vi "Configure Session.vi"(8 "error in":errorcluster, 11 "Plugin in":refnum<class "Nominal-TDMS-Upload.lvclass">) -> (0 "error out":errorcluster, 3 "Plugin out":refnum<class "Nominal-TDMS-Upload.lvclass">)   [LabVIEW 2026, in "Nominal-TDMS-Upload.lvlib" / "Nominal-TDMS-Upload.lvclass"]
uses:
  Nominal-TDMS-Upload.lvclass
  C:/Program Files/National Instruments/LabVIEW 2026/vi.lib/FlexLogger/SDK/PluginSDK.lvlibp/PEFClasses/SDK/Plugin/Plugin.lvclass
  stream reference data.ctl
  <vilib>/Nominal/Nominal IO Client/lv_src/Nominal Client/Nominal Client.lvclass
  <vilib>/Nominal/Nominal IO Client/lv_src/datasources/dataset/dataset.lvclass
  <vilib>/Nominal/Nominal IO Client/submodules/nominal-streaming-labview-ffi/lv_src/Stream/Stream.lvclass
  <vilib>/Nominal/Nominal IO Client/submodules/nominal-streaming-labview-ffi/lv_src/Channel/Channel.lvclass
  <vilib>/Nominal/Nominal IO Client/lv_src/Nominal Client/Nominal Client.lvclass/Nominal Client.ctl
  Nominal-TDMS-Upload.lvclass/Nominal-TDMS-Upload.ctl
  04996bb8-e45a-4ac7-aa6a-ac4592b39374.vi
  <vilib>/Nominal/Nominal IO Client/lv_src/Nominal Client/private_data.set.vi
  04996bb8-e45a-4ac7-aa6a-ac4592b39374.vi/8284acbc-2d4d-4b18-b492-8ff51a6e7e10.vi
  <vilib>/Nominal/Nominal IO Client/lv_src/Nominal Client/Palette Items/destroy.vi
  <vilib>/Nominal/Nominal IO Client/lv_src/nominal types/workspace/id.get.vi
  <vilib>/Nominal/Nominal IO Client/lv_src/nominal types/workspace/rid.get.vi
  <vilib>/AdvancedString/1D String Array to Delimited String.vi
  <vilib>/Nominal/Nominal IO Client/lv_src/Nominal Client/workspace.set.vi
  <vilib>/FlexLogger/SDK/PluginSDK.lvlibp/PEFClasses/SDK/Plugin/ParameterAccess/Read String.vi
  async convert file.vi
  <vilib>/Utility/file.llb/Application Directory.vi
  <vilib>/Nominal/Nominal IO Client/lv_src/Nominal Client/format endpoint termination.vi
  <vilib>/Nominal/Nominal IO Client/submodules/reqwest-labview/lv-src/reqwest/create.vi
  <vilib>/Nominal/Nominal IO Client/lv_src/Nominal Client/workspace_cache.get_from_rid.vi
  <vilib>/Nominal/Nominal IO Client/lv_src/Nominal Client/workspace_cache.get.vi
  <vilib>/Nominal/Nominal IO Client/lv_src/Nominal Client/Palette Items/who_am_i.vi
  <vilib>/Nominal/Nominal IO Client/submodules/reqwest-labview/lv-src/reqwest/destroy.vi
  <vilib>/Nominal/Nominal IO Client/lv_src/User/User.lvclass
  <vilib>/Nominal/Nominal IO Client/lv_src/nominal types/workspace/workspace.lvclass
  <vilib>/Nominal/Nominal IO Client/submodules/reqwest-labview/lv-src/reqwest/reqwest.lvclass
  <vilib>/FlexLogger/SDK/PluginSDK.lvlibp/PEFClasses/SDK/Message Completion Handler/Message Completion Handler.lvclass
  C:/Program Files/National Instruments/LabVIEW 2026/vi.lib/FlexLogger/SDK/PluginSDK.lvlibp/PEFClasses/SDK/Processing Element/Processing Element.lvclass
  C:/sw/ni-flexlogger-streaming-plugin/Nominal-TDMS-Upload/Nominal-TDMS-Upload.lvclass
  <vilib>/FlexLogger/SDK/PluginSDK.lvlibp/PEFClasses/SDK/Plugin/Plugin.lvclass
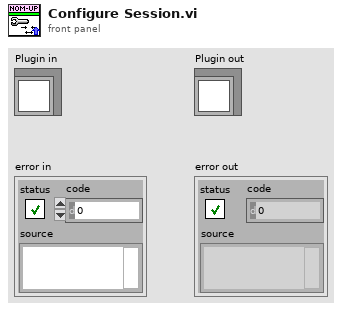
[diagram p1: front panel]
types:
  T1 = typedef "Nominal-TDMS-Upload.lvlib/Nominal-TDMS-Upload.lvclass/stream reference data.ctl" = cluster{"Nominal Client":refnum<class "Nominal Client.lvclass">, "Dataset":refnum<class "dataset.lvclass">, "dataset stream":refnum<class "Stream.lvclass">, "Map":map{string, refnum<class "Channel.lvclass">}}
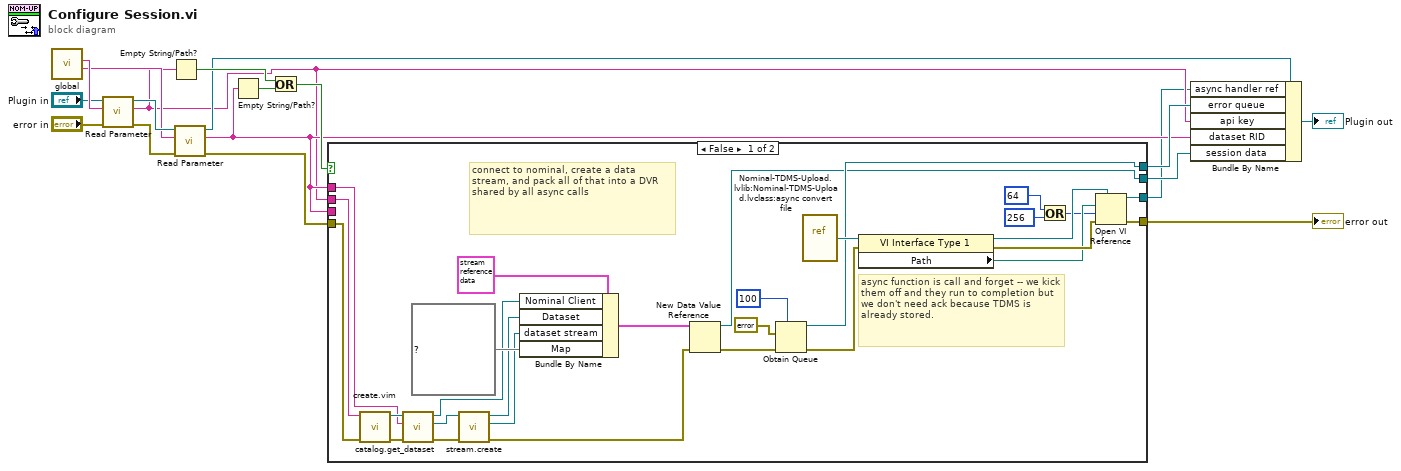
[diagram p0: block diagram]
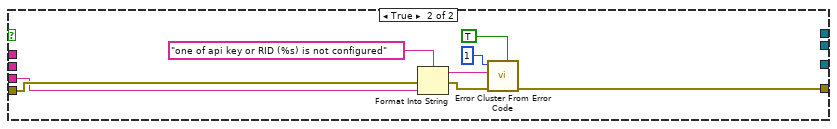
[diagram p2: hidden frame]
diagram:
  n1 = call "global.vi"() -> ("dataset RID"=w10:string, "API Key"=w11:string)  [unwired: 9 in, 1 out]
  n2 = call-poly <vilib>:"Read Parameter.vi"("error in (no error)"="error in", "Name"=w11, "Plugin in"="Plugin in") -> ("error out"=w14:errorcluster, "Value"=w3:string, "Plugin out"=w15:refnum<class "Nominal-TDMS-Upload.lvclass">)  [unwired: 5 in, 1 out]
  n3 = Empty String/Path?(string/path=w3) -> (empty?=w12:bool)
  n4 = call-poly <vilib>:"Read Parameter.vi"("error in (no error)"=w14, "Name"=w10, "Plugin in"=w15) -> ("error out"=w6:errorcluster, "Value"=w4:string, "Plugin out"=w8:refnum<class "Nominal-TDMS-Upload.lvclass">)  [unwired: 5 in, 1 out]
  n5 = Empty String/Path?(string/path=w4) -> (empty?=w13:bool)
  n6 = Or(x=w12, y=w13) -> (x .or. y?=w5:bool)
  n7 = case shown="False" w5 {
    tunnel: [w37 _] -> w1
    tunnel: [w36 _] -> w17
    tunnel: [w33 w54] -> w16
    tunnel: w6 -> [w35 w55]
    tunnel: w4 -> [_ w50]
    tunnel: w4 -> [w30 _]
    tunnel: w3 -> [w29 _]
    tunnel: [w24 _] -> w2
    frame False {
      # "async function is call and forget -- we kick them off and they run to completion but we don't need ack because TDMS is already stored."
      # "connect to nominal, create a data stream, and pack all of that into a DVR shared by all async calls"
      n8 = call "create.vim"("error in"=w35, "API Token (string or path)"=w29) -> ("error out"=w32:errorcluster, "Nominal Client"=w34:refnum<class "Nominal Client.lvclass">)  [unwired: 7 in, 1 out]
      n9 = call <vilib>:"catalog.get_dataset.vi"("error in"=w32, "Dataset RID"=w30, "Nominal Client in"=w34) -> ("error out"=w31:errorcluster, "Dataset"=w28:refnum<class "dataset.lvclass">, "Nominal Client out"=w19:refnum<class "Nominal Client.lvclass">)  [unwired: 6 in]
      n10 = call <vilib>:"stream.create.vi"("error in (no error)"=w31, "dataset in"=w28) -> ("error out"=w26:errorcluster, "Stream"=w21:refnum<class "Stream.lvclass">, "dataset out"=w20:refnum<class "dataset.lvclass">)  [unwired: 7 in]
      n11 = Bundle By Name(cluster=T1 {"Nominal Client"=refnum, "Dataset"=refnum, "dataset stream"=refnum, "Map"={}} ("stream channels"), "Nominal Client"=w19, "Dataset"=w20, "dataset stream"=w21, "Map"=map{string, refnum<class "Channel.lvclass">} {}) -> (w23:T1)
      n12 = New Data Value Reference(data value=w23, error in=w26) -> (data value reference=w24:refnum<data-value>, error out=w25:errorcluster)
      n13 = Obtain Queue(max queue size (-1, unlimited)=100, element data type=errorcluster {"status"=FALSE, "code"=0, "source"=""} ("error in (no error)"), error in (no error)=w25) -> (queue out=w36:refnum<queue>, error out=w40:errorcluster)  [unwired: 2 in, 1 out]
      n14 = vi-ref "Nominal-TDMS-Upload.lvlib:Nominal-TDMS-Upload.lvclass:async convert file.vi"() -> (w47:refnum<vi>)
      n15 = property class="VI Interface Type 1"(reference=w47, error in=w40) -> (reference out=w44:refnum<vi>, error out=w46:errorcluster, "Path"=w45:path)
      n16 = Or(x=64 ("options"), y=256 ("options")) -> (x .or. y?=w42:i32)
      n17 = Open VI Reference(type specifier VI Refnum (for type only)=w44, vi path=w45, options=w42, error in (no error)=w46) -> (vi reference=w37:refnum<vi>, error out=w33:errorcluster)  [unwired: 2 in]
    }
    frame True {
      n18 = Format Into String(format string="one of api key or RID (%s) is not configured", error in=w55, w50) -> (resulting string=w51:string, error out=w52:errorcluster)  [unwired: 1 in]
      n19 = call <vilib>:"Error Cluster From Error Code.vi"("is warning? (False)"=TRUE, "error in (no error)"=w52, "error message (\"\")"=w51, "error code (0)"=1) -> ("error out"=w54:errorcluster)  [unwired: 5 in]
    }
  }
  "error out" <- w16
  n20 = Bundle By Name(cluster=w8, "async handler ref"=w1, "error queue"=w17, "api key"=w3, "dataset RID"=w4, "session data"=w2) -> (→"Plugin out":refnum<class "Nominal-TDMS-Upload.lvclass">)
